vi "query Start and Stop Frequency.vi"(8 "error in (no error)":errorcluster, 11 "FSV-40N in":refnum<class "FSV-40N.lvclass">) -> (0 "error out":errorcluster, 2 "Start/Stop Frequency(Hz)":T1 {"Stop" format="%#_6p"; "Start" format="%#_6p"}, 3 "FSV-40N out":refnum<class "FSV-40N.lvclass">)   [LabVIEW 2023, in "Spectrum Analyzer.lvlib" / "FSV-40N.lvclass"]
uses:
  FSV-40N.lvclass
  FSV-40N.lvclass/FSV-40N.ctl
  Spectrum Analyzer.lvlib
  TYPE DEFINITION/TYPE Start and Stop Frequency.ctl
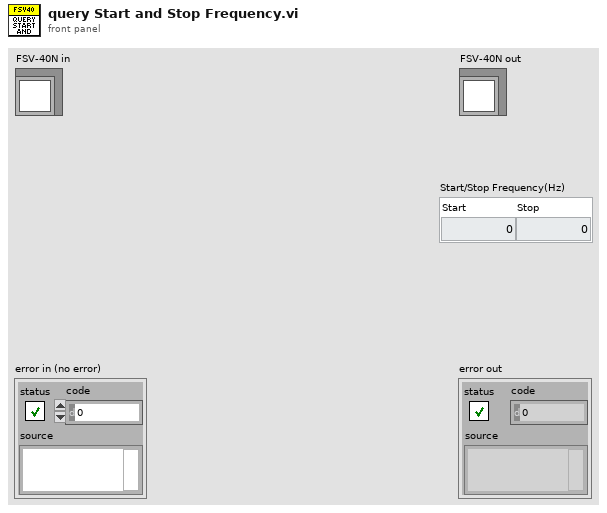
[diagram p1: front panel]
types:
  T1 = typedef "Spectrum Analyzer.lvlib/TYPE Start and Stop Frequency.ctl" = cluster{"Start":dbl, "Stop":dbl}
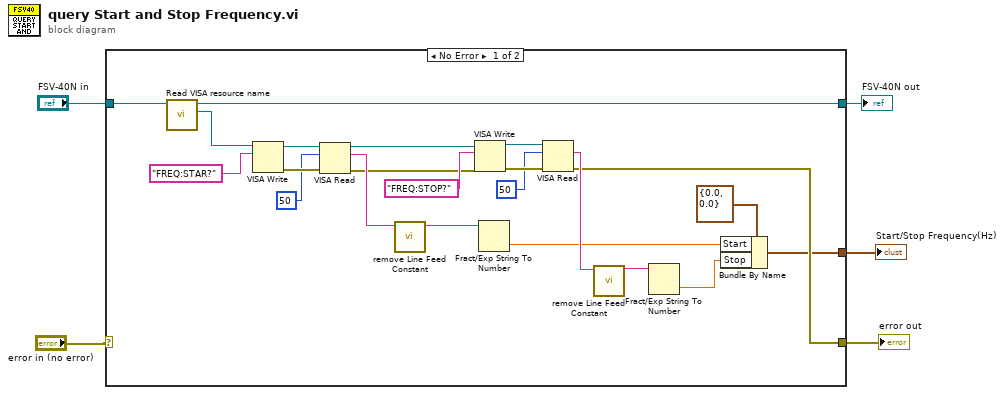
[diagram p0: block diagram]
diagram:
  n1 = case shown="No Error" "error in (no error)" {
    selector: "error in (no error)" -> [_ w29]
    tunnel: "FSV-40N in" -> [w27 w28]
    tunnel: [w12 w29] -> w1
    tunnel: [w23 w28] -> w4
    tunnel: [w6 _] -> w3
    frame No Error {
      n2 = call "Read VISA resource name.vi"("FSV-40N in"=w27) -> ("VISA resource name"=w26:refnum<visa-resource-name>, "FSV-40N out"=w23:refnum<class "FSV-40N.lvclass">)  [unwired: 8 in, 1 out]
      n3 = VISA Write(VISA resource name=w26, write buffer="FREQ:STAR?") -> (VISA resource name out=w22:refnum<visa-resource-name>, error out=w21:errorcluster)  [unwired: 1 in, 1 out]
      n4 = VISA Read(VISA resource name=w22, byte count=u32 50, error in (no error)=w21) -> (VISA resource name out=w18:refnum<visa-resource-name>, read buffer=w19:string, error out=w17:errorcluster)  [unwired: 1 out]
      n5 = call "remove Line Feed Constant.vi"("Input String"=w19) -> ("Line Feed Removed String"=w11:string)  [unwired: 10 in]
      n6 = VISA Write(VISA resource name=w18, write buffer="FREQ:STOP?", error in (no error)=w17) -> (VISA resource name out=w16:refnum<visa-resource-name>, error out=w15:errorcluster)  [unwired: 1 out]
      n7 = Fract/Exp String To Number(string=w11) -> (number=w9:dbl)  [unwired: 3 in, 1 out]
      n8 = VISA Read(VISA resource name=w16, byte count=u32 50, error in (no error)=w15) -> (read buffer=w13:string, error out=w12:errorcluster)  [unwired: 2 out]
      n9 = call "remove Line Feed Constant.vi"("Input String"=w13) -> ("Line Feed Removed String"=w8:string)  [unwired: 10 in]
      n10 = Fract/Exp String To Number(string=w8) -> (number=w7:dbl)  [unwired: 3 in, 1 out]
      n11 = Bundle By Name(cluster=T1 {"Start"=0.0, "Stop"=0.0} ("Start/Stop Frequency(Hz) 2"), "Start"=w9, "Stop"=w7) -> (w6:T1)
    }
    frame Error {
    }
  }
  "error out" <- w1
  "FSV-40N out" <- w4
  "Start/Stop Frequency(Hz)" <- w3
